vi "disable stepper.vi"(8 "error in (no error)":errorcluster, 10 "Disable Stepper (T)":bool=TRUE, 11 "CL57RS in":refnum<class "CL57RS.lvclass">) -> (0 "error out":errorcluster, 3 "CL57RS out":refnum<class "CL57RS.lvclass">)   [LabVIEW 2025, in "Motor.lvlib" / "CL57RS.lvclass"]
uses:
  CL57RS.lvclass
  CL57RS.lvclass/CL57RS.ctl
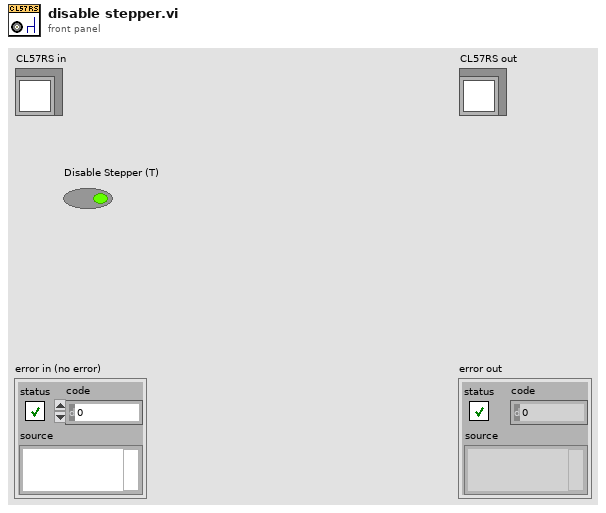
[diagram p1: front panel]
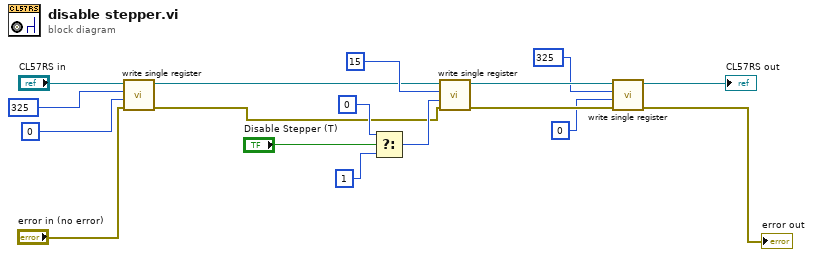
[diagram p0: block diagram]
diagram:
  n1 = call "write single register.vi"("error in (no error)"="error in (no error)", "register to write"=u16 0 ("address"), "address"=u16 325, "CL57RS in"="CL57RS in") -> ("error out"=w8:errorcluster, "CL57RS out"=w12:refnum<class "CL57RS.lvclass">)  [unwired: 6 in]
  n2 = Select(t=u16 0 ("address"), s="Disable Stepper (T)", f=u16 1 ("address")) -> (s? t:f=w13:u16)
  n3 = call "write single register.vi"("error in (no error)"=w8, "register to write"=w13, "address"=u16 15, "CL57RS in"=w12) -> ("error out"=w4:errorcluster, "CL57RS out"=w5:refnum<class "CL57RS.lvclass">)  [unwired: 6 in]
  n4 = call "write single register.vi"("error in (no error)"=w4, "register to write"=u16 0 ("address"), "address"=u16 325, "CL57RS in"=w5) -> ("error out"=→"error out":errorcluster, "CL57RS out"=→"CL57RS out":refnum<class "CL57RS.lvclass">)  [unwired: 6 in]
